vi "Footer.vi"() -> ()   [LabVIEW 2013]
uses:
  <vilib>/Utility/miscctls.llb/LVPointTypeDef.ctl
  Globals/Global VI.vi
panel:
  in  "Last Button":bool
  in  "Next Button":bool
  in  "First Button":bool
  in  "Previous Button":bool
  in  "Cluster":T1
  out "array":bool[](array[boolean])
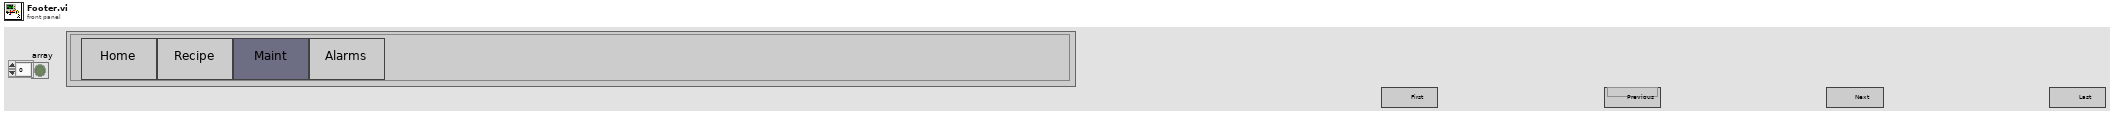
[diagram p1: front panel]
types:
  T1 = cluster{"OK Button":bool, "OK Button 2":bool, "OK Button 3":bool, "OK Button 4":bool, "OK Button 5":bool, "OK Button 6":bool, "OK Button 7":bool, "OK Button 8":bool, "OK Button 9":bool, "OK Button 10":bool, "OK Button 11":bool, "OK Button 12":bool, "OK Button 13":bool}
  T2 = typedef "LVPointTypeDef.ctl" = cluster{"Horizontal":i16, "Vertical":i16}
  T3 = enum16{"Always On", "Always Off", "Off While Running"}
  T4 = typedef "LVAllMonitorsDisplayTypeDef.ctl" = cluster{"Bounds":cluster{"Left":i16, "Top":i16, "Right":i16, "Bottom":i16}, "Depth":i16}[]
  T5 = typedef "LVRectTypeDef.ctl" = cluster{"Left":i16, "Top":i16, "Right":i16, "Bottom":i16}
  T6 = cluster{"Bounds":cluster{"Left":i16, "Top":i16, "Right":i16, "Bottom":i16}, "Depth":i16}
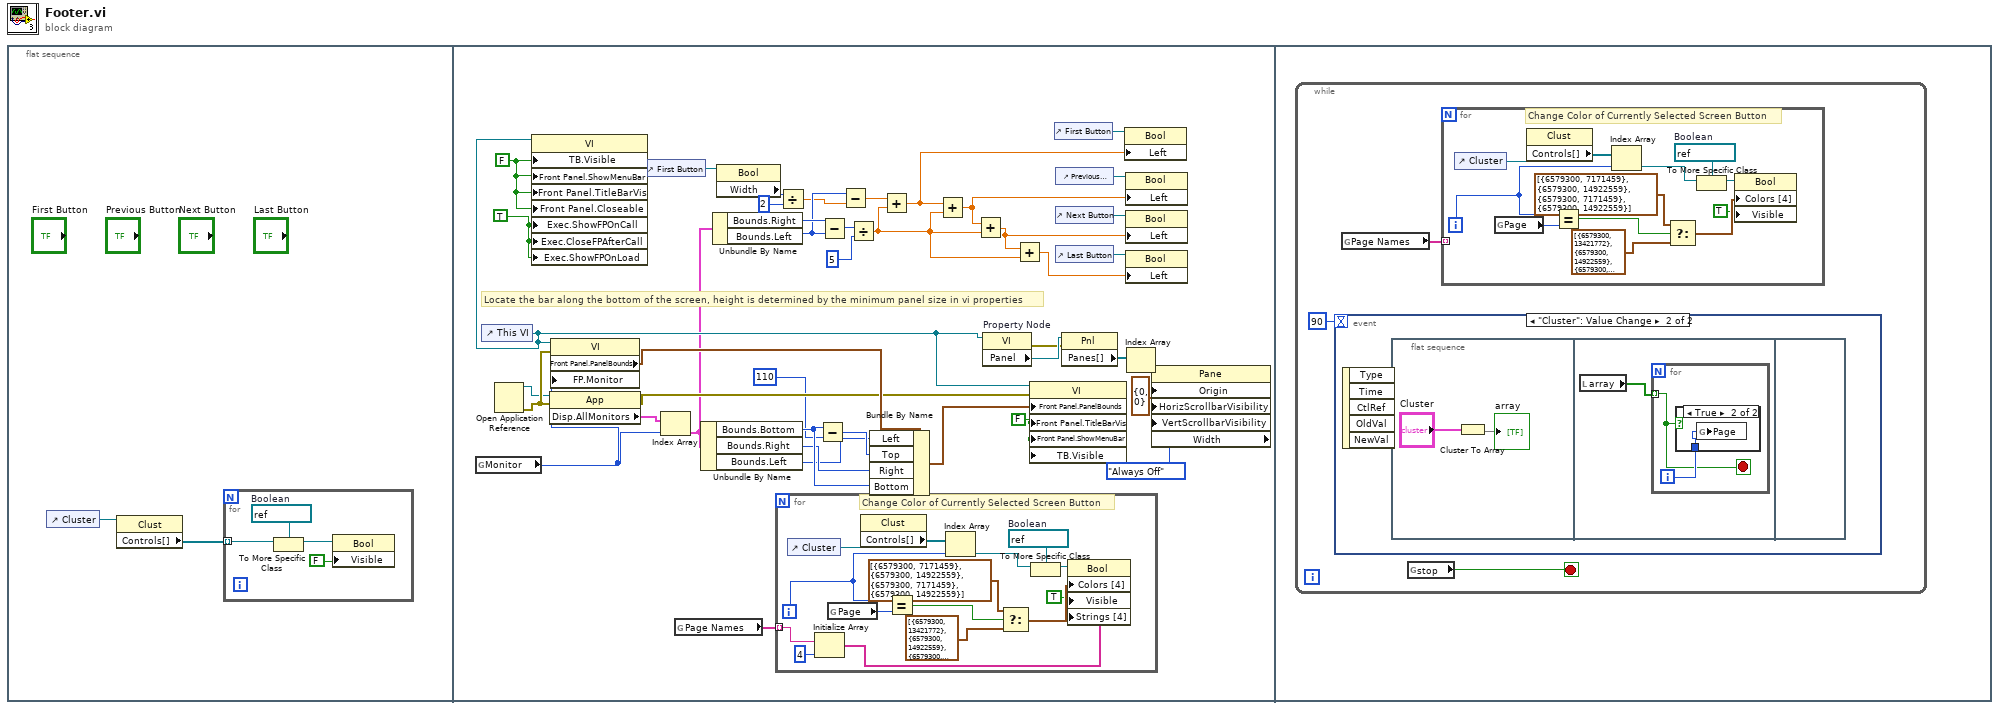
[diagram p0: block diagram]
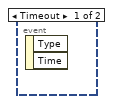
[diagram p2: hidden frame]
diagram:
  n1 = flat-sequence {
    frame #0 {
      n2 = control-ref of="Cluster"() -> (w1:refnum<vi>)
      n3 = property class="Clust"(reference=w1) -> ("Controls[]"=w2:refnum<vi>[])  [unwired: 1 in, 2 out]
      n4 = for {
        tunnel: w2 -> [w3] mode=indexing
        w4 = refnum<vi> refnum  # Boolean
        n5 = To More Specific Class(target class=w4, reference=w3) -> (specific class reference=w5:refnum<vi>)  [unwired: 1 in, 1 out]
        n6 = property class="Bool"(reference=w5, "Visible"=FALSE) -> ()  [unwired: 1 in, 2 out]
      }
    }
    frame #1 {
      w31 = TRUE ("Execution:Show Front Panel On Call")
      w30 = FALSE ("Tool Bar:Visible")
      w32 = T3."Always Off" ("Horizontal Scrollbar Visibility")
      w34 = FALSE ("Front Panel Window:Title Bar Visible")
      # "Locate the bar along the bottom of the screen, height is determined by the minimum panel size in vi properties"
      n7 = global read "Global VI.vi" "Monitor"() -> (w33:u16)
      n8 = control-ref of="This VI"() -> (w29:refnum<vi>)
      n9 = Open Application Reference() -> (0:w48:errorcluster, 3:w47:refnum<vi>)  [unwired: 4 in]
      n10 = property class="VI"(reference=w29, "TB.Visible"=w30, "Front Panel.ShowMenuBar"=w30, "Front Panel.TitleBarVis"=w30, "Front Panel.Closeable"=w30, "Exec.ShowFPOnCall"=w31, "Exec.CloseFPAfterCall"=w31, "Exec.ShowFPOnLoad"=w31) -> ()  [unwired: 1 in, 2 out]
      n11 = property class="App"(reference=w47, error in=w48) -> (error out=w42:errorcluster, "Disp.AllMonitors"=w41:T4)  [unwired: 1 out]
      n12 = property class="VI"(reference=w29, error in=w48, "FP.Monitor"=w33) -> ("Front Panel.PanelBounds"=w44:T5)  [unwired: 2 out]
      n13 = control-ref of="First Button"() -> (w13:refnum<vi>)
      n14 = Index Array(array=w41, index=w33) -> (element=w22:T6)
      n15 = global read "Global VI.vi" "Page Names"() -> (w7:string[])
      n16 = Unbundle By Name(w22) -> ("Bounds.Bottom"=w46:i16, "Bounds.Right"=w28:i16, "Bounds.Left"=w27:i16)
      n17 = Unbundle By Name(w22) -> ("Bounds.Right"=w21:i16, "Bounds.Left"=w10:i16)
      n18 = property class="Bool"(reference=w13) -> ("Width"=w12:u32)  [unwired: 1 in, 2 out]
      n19 = for {
        tunnel: w7 -> [w51] mode=indexing
        i -> [w57]
        w63 = refnum<vi> refnum  # Boolean
        # "Change Color of Currently Selected Screen Button"
        n20 = control-ref of="Cluster"() -> (w59:refnum<vi>)
        n21 = Initialize Array(w51, 4 ("dimension size")) -> (w49:string[])
        n22 = global read "Global VI.vi" "Page"() -> (w58:i16)
        n23 = property class="Clust"(reference=w59) -> ("Controls[]"=w61:refnum<vi>[])  [unwired: 1 in, 2 out]
        n24 = Equal?(x=w57, y=w58) -> (x = y?=w56:bool)
        n25 = Index Array(array=w61, index=w57) -> (element=w60:refnum<vi>)
        n26 = Select(t=cluster{u32, u32}[] [{6579300, 7171459}, {6579300, 14922559}, {6579300, 7171459}, {6579300, 14922559}] ("Colors [4]"), s=w56, f=cluster{u32, u32}[] [{6579300, 13421772}, {6579300, 14922559}, {6579300, 13421772}, {6579300, 14922559}] ("Colors [4]")) -> (s? t:f=w54:cluster{u32, u32}[])
        n27 = To More Specific Class(target class=w63, reference=w60) -> (specific class reference=w62:refnum<vi>)  [unwired: 1 in, 1 out]
        n28 = property class="Bool"(reference=w62, "Colors [4]"=w54, "Visible"=TRUE, "Strings [4]"=w49) -> ()  [unwired: 1 in, 2 out]
      }
      n29 = Divide(x=w12, y=u32 2) -> (x/y=w9:dbl)
      n30 = Subtract(x=w46, y=i16 110) -> (x-y=w45:i16)
      n31 = Subtract(x=w21, y=w10) -> (x-y=w20:i16)
      n32 = Subtract(x=w10, y=w9) -> (x-y=w8:dbl)
      n33 = Divide(x=w20, y=i16 5) -> (x/y=w15:dbl)
      n34 = Bundle By Name(cluster=w44, "Left"=w27, "Top"=w45, "Right"=w28, "Bottom"=w46) -> (w43:T5)
      n35 = Add(x=w8, y=w15) -> (x+y=w18:dbl)
      n36 = Add(x=w18, y=w15) -> (x+y=w17:dbl)
      n37 = Add(x=w17, y=w15) -> (x+y=w16:dbl)
      n38 = property on="Property Node" class="VI"(reference=w29) -> (error out=w39:errorcluster, "Panel"=w40:refnum<vi>)  [unwired: 1 in, 1 out]
      n39 = Add(x=w16, y=w15) -> (x+y=w14:dbl)
      n40 = property class="VI"(reference=w29, error in=w42, "Front Panel.PanelBounds"=w43, "Front Panel.TitleBarVis"=w34, "Front Panel.ShowMenuBar"=w34, "TB.Visible"=w34) -> ()  [unwired: 2 out]
      n41 = control-ref of="First Button"() -> (w23:refnum<vi>)
      n42 = control-ref of="Previous Button"() -> (w24:refnum<vi>)
      n43 = control-ref of="Next Button"() -> (w25:refnum<vi>)
      n44 = control-ref of="Last Button"() -> (w26:refnum<vi>)
      n45 = property class="Pnl"(reference=w40, error in=w39) -> ("Panes[]"=w38:refnum<vi>[])  [unwired: 2 out]
      n46 = property class="Bool"(reference=w23, "Left"=w18) -> ()  [unwired: 1 in, 2 out]
      n47 = property class="Bool"(reference=w24, "Left"=w17) -> ()  [unwired: 1 in, 2 out]
      n48 = property class="Bool"(reference=w25, "Left"=w16) -> ()  [unwired: 1 in, 2 out]
      n49 = property class="Bool"(reference=w26, "Left"=w14) -> ()  [unwired: 1 in, 2 out]
      n50 = Index Array "Index Array"(array=w38) -> (element=w37:refnum<vi>)  [unwired: 1 in]
      n51 = property class="Pane" props=["Origin", "HorizScrollbarVisibility", "VertScrollbarVisibility", "Width"](reference=w37, "Origin"=T2 {"Horizontal"=0, "Vertical"=0}, "HorizScrollbarVisibility"=w32, "VertScrollbarVisibility"=w32) -> ()  [unwired: 1 in, 3 out]
    }
    frame #2 {
      n52 = while {
        stop <- w65 stop-if-true
        n53 = event shown="[1] \"Cluster\": Value Change" {
          selector: _ -> [_ _]
          dyn-events: _ -> [_ _]
          timeout: 90 -> [_ _]
          event Timeout {
            n54 = event-data() -> ()  [unwired: 1 in, 2 out]
          }
          event "Cluster": Value Change {
            n55 = event-data() -> ()  [unwired: 1 in, 5 out]
            n56 = flat-sequence {
              frame #0 {
                n57 = Cluster To Array(cluster="Cluster") -> (array=→"array":bool[])
              }
              frame #1 {
                n58 = local read "array"() -> (w81:bool[])
                n59 = for {
                  tunnel: w81 -> [w82] mode=indexing
                  i -> [w83]
                  stop <- w82 stop-if-true
                  n60 = case shown="True" w82 {
                    tunnel: w83 -> [_ w84]
                    frame False {
                    }
                    frame True {
                      n61 = global write "Global VI.vi" "Page"(w84) -> ()
                    }
                  }
                }
              }
              frame #2 {
              }
            }
          }
        }
        n62 = global read "Global VI.vi" "Page Names"() -> (w64:string[])
        n63 = global read "Global VI.vi" "stop"() -> (w65:bool)
        n64 = for {
          tunnel: w64 -> [_] mode=indexing
          i -> [w72]
          w78 = refnum<vi> refnum  # Boolean
          # "Change Color of Currently Selected Screen Button"
          n65 = control-ref of="Cluster"() -> (w74:refnum<vi>)
          n66 = global read "Global VI.vi" "Page"() -> (w73:i16)
          n67 = property class="Clust"(reference=w74) -> ("Controls[]"=w76:refnum<vi>[])  [unwired: 1 in, 2 out]
          n68 = Equal?(x=w72, y=w73) -> (x = y?=w71:bool)
          n69 = Index Array(array=w76, index=w72) -> (element=w75:refnum<vi>)
          n70 = Select(t=cluster{u32, u32}[] [{6579300, 7171459}, {6579300, 14922559}, {6579300, 7171459}, {6579300, 14922559}] ("Colors [4]"), s=w71, f=cluster{u32, u32}[] [{6579300, 13421772}, {6579300, 14922559}, {6579300, 13421772}, {6579300, 14922559}] ("Colors [4]")) -> (s? t:f=w69:cluster{u32, u32}[])
          n71 = To More Specific Class(target class=w78, reference=w75) -> (specific class reference=w77:refnum<vi>)  [unwired: 1 in, 1 out]
          n72 = property class="Bool"(reference=w77, "Colors [4]"=w69, "Visible"=TRUE) -> ()  [unwired: 1 in, 2 out]
        }
      }
    }
  }
